vi "libssh2_sftp_rename_ex.vi"(7 "flags":i32(ring) items=["Overwrite"=1, "Atomic"=2, "Native"=4], 8 "error in (no error)":errorcluster, 9 "destination file":string, 10 "source file":string, 11 "sftp":T1) -> (0 "error out":errorcluster)   [LabVIEW 2017, in "libssh2.lvlib"]
doc: "Rename a file or directory with custom flags.\n\nCreates a hard link to the file or directory at the new location and then removes the original file or directory.\n\n<B>Remarks</B>\nServices that watch for file changes may not detect the rename operation. Use <B>libssh2_sftp_posix_rename_ex</B> for a true rename operation."
uses:
  libssh2.lvlib
  SFTP Refnum.ctl
  Acquire Session.vi
  Release Session.vi
  Not An SFTP Refnum.vi
  <vilib>/Utility/error.llb/Error Cluster From Error Code.vi
  Global Settings.vi
  Read SFTP Refnum.vi
  Read Session Refnum.vi
  <vilib>/Utility/semaphor.llb/Acquire Semaphore.vi
  <vilib>/Utility/semaphor.llb/Release Semaphore.vi
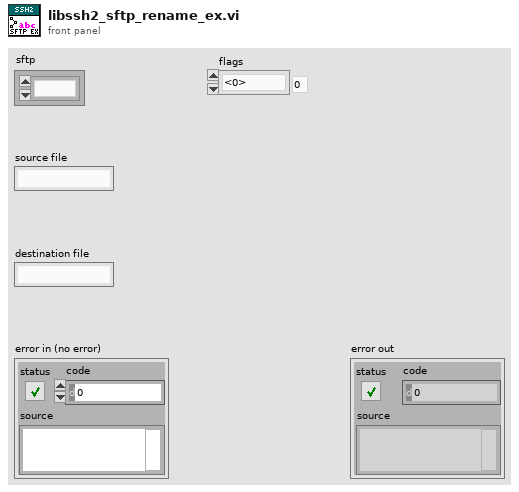
[diagram p1: front panel]
types:
  T1 = typedef "libssh2.lvlib/SFTP Refnum.ctl" = refnum<k1>
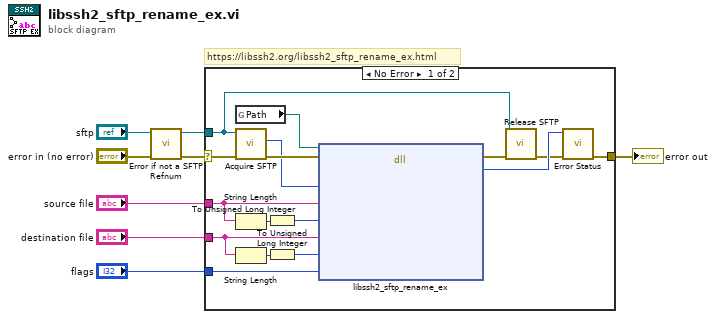
[diagram p0: block diagram]
diagram:
  # "https://libssh2.org/libssh2_sftp_rename_ex.html"
  n1 = call "Error if not a SFTP Refnum.vi"("error in (no error)"="error in (no error)", "sftp"="sftp") -> ("error out"=w7:errorcluster, "sftp out"=w6:T1)  [unwired: 8 in]
  n2 = case shown="No Error" w7 {
    selector: w7 -> [w23 w25]
    tunnel: w6 -> [w9 _]
    tunnel: [w19 w25] -> w5
    tunnel: "source file" -> [w17 _]
    tunnel: "flags" -> [w14 _]
    tunnel: "destination file" -> [w11 _]
    frame No Error {
      n3 = global read "Global Settings.vi" "Path"() -> (w24:path)
      n4 = call "Acquire SFTP.vi"("error in (no error)"=w23, "sftp"=w9) -> ("error out"=w22:errorcluster, "LIBSSH2_SFTP*"=w21:u64)  [unwired: 8 in]
      n5 = String Length(string=w17) -> (length=w16:i32)
      n6 = String Length(string=w11) -> (length=w13:i32)
      n7 = To Unsigned Long Integer(number=w16) -> (unsigned 32bit integer=w15:u32)
      n8 = To Unsigned Long Integer(number=w13) -> (unsigned 32bit integer=w12:u32)
      n9 = dll-call lib="?" fn="libssh2_sftp_rename_ex"(path in=w24, error in=w22, "sftp"=w21, "source_filename"=w17, "source_filename_len"=w15, "dest_filename"=w11, "dest_filename_len"=w12, "flags"=w14) -> (error out=w20:errorcluster, "return value"=w18:i32)  [unwired: 7 in, 1 out]
      n10 = call "Release SFTP.vi"("error in (no error)"=w20, "sftp"=w9) -> ("error out"=w10:errorcluster)  [unwired: 9 in]
      n11 = call "Error Status.vi"("error in (no error)"=w10, "return value"=w18) -> ("error out"=w19:errorcluster)  [unwired: 8 in, 1 out]
    }
    frame Error {
    }
  }
  "error out" <- w5
